vi "RDB Compose Message.vi"(8 "error in (no error)":errorcluster, 10 "RDB Reference in":T4, 11 "Settings in":T1={"UDP Receiver"=refnum, "UDP Sender"=refnum, "Valid Packet"=FALSE, "TCP"=refnum, "Network Settings"={"IP adress"="127.0.0.1", "RDB"={"Protocol"=enum."UDP", "Tx Port"=48270, "Rx Port"=10, "Buffer Size"=204800, "Timeout"=10}, "SCP"={"Protocol"=enum."TCP", "Tx Port"=48191, "Rx Port"=48191, "Buffer Size"=204800, "Timeout"=10}}, "vclient"=path "", "paeseHandle"=0, "builderHandle"=0}) -> (0 "error out":errorcluster, 2 "RDB Reference out":T4, 3 "Settings out":T1={"UDP Receiver"=refnum, "UDP Sender"=refnum, "Valid Packet"=FALSE, "TCP"=refnum, "Network Settings"={"IP adress"="127.0.0.1", "RDB"={"Protocol"=enum."UDP", "Tx Port"=48270, "Rx Port"=10, "Buffer Size"=204800, "Timeout"=10}, "SCP"={"Protocol"=enum."TCP", "Tx Port"=48191, "Rx Port"=48191, "Buffer Size"=204800, "Timeout"=10}}, "vclient"=path "", "paeseHandle"=0, "builderHandle"=0})   [LabVIEW 2023, in "RDB.lvlib"]
uses:
  RDB.lvlib
  RDB References.ctl
  DataContainer/DataContainer.lvclass
  Engine/Type/Settings.ctl
  Shared/Network Settings.ctl
  Shared/Protocol.ctl
  Shared/Vires VTD Shared.lvlib
  Engine/Vires VTD Engine.lvlib
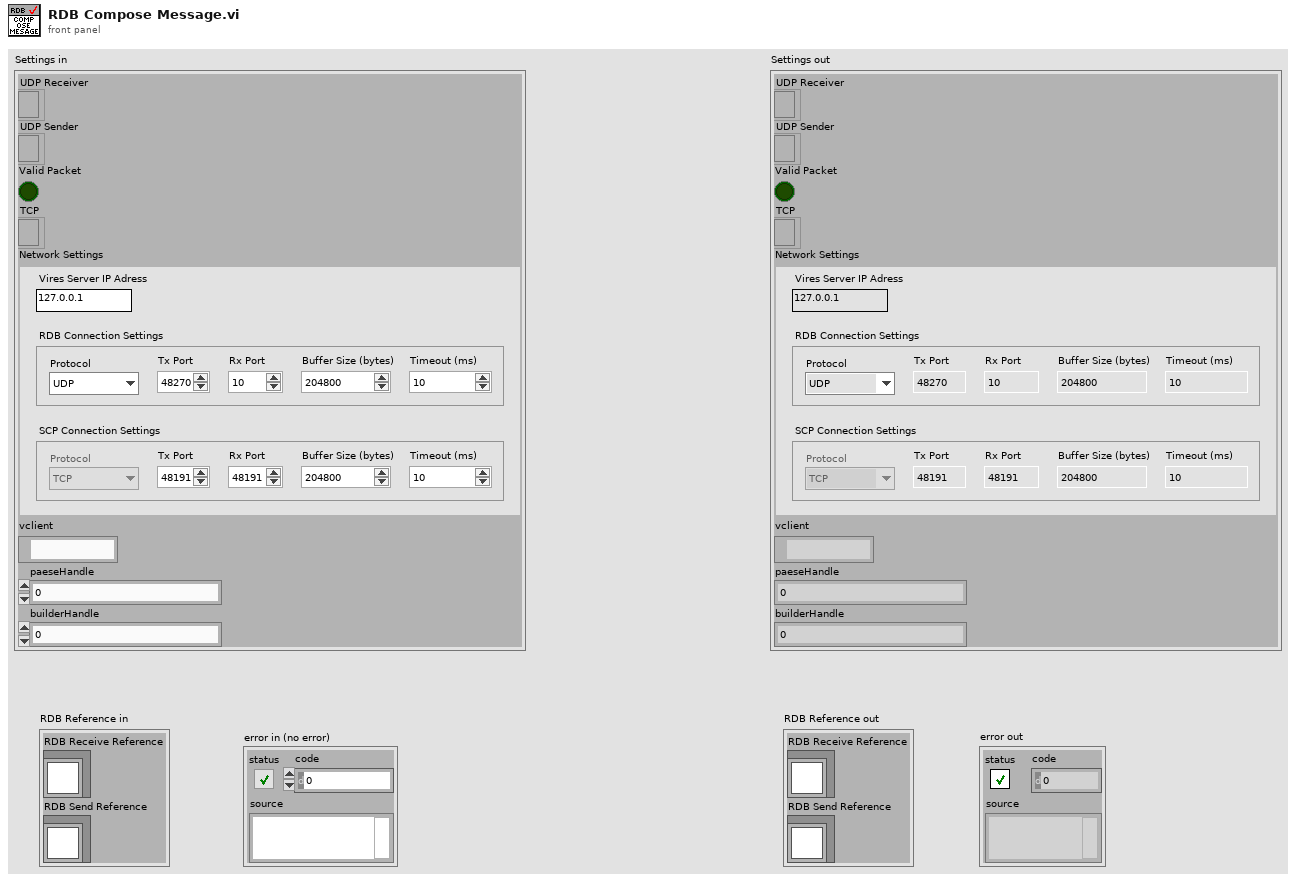
[diagram p1: front panel]
types:
  T1 = typedef "Vires VTD Engine.lvlib/Settings.ctl" = cluster{"UDP Receiver":refnum<k16>, "UDP Sender":refnum<k16>, "Valid Packet":bool, "TCP":refnum<k5>, "Network Settings":T2, "vclient":path, "paeseHandle":u64, "builderHandle":u64}
  T2 = typedef "Vires VTD Shared.lvlib/Network Settings.ctl" = cluster{"IP adress":string, "RDB":cluster{"Protocol":T3, "Tx Port":u16, "Rx Port":u16, "Buffer Size":i32, "Timeout":u16}, "SCP":cluster{"Protocol":T3, "Tx Port":u16, "Rx Port":u16, "Buffer Size":i32, "Timeout":u16}}
  T3 = typedef "Vires VTD Shared.lvlib/Protocol.ctl" = enum16{"UDP", "TCP"}
  T4 = typedef "RDB.lvlib/RDB References.ctl" = cluster{"RDB Receive Reference":refnum<class "DataContainer.lvclass">, "RDB Send Reference":refnum<class "DataContainer.lvclass">}
  T5 = typedef "XNET Frame FlexRay.ctl" = cluster{"timestamp":timestamp, "payload":u8[], "slot":u16, "type":T6, "cycle count":u8, "startup?":bool, "sync?":bool, "preamble?":bool, "ch A":bool, "ch B":bool, "echo?":bool}
  T6 = typedef "XNET Frame Type FlexRay.ctl" = u8
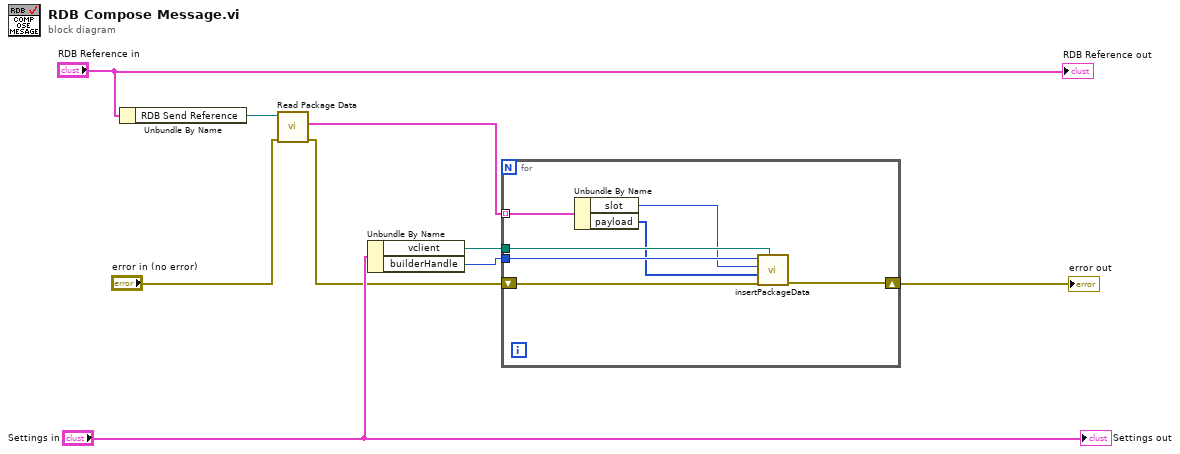
[diagram p0: block diagram]
diagram:
  n1 = Unbundle By Name("RDB Reference in") -> ("RDB Send Reference"=w4:refnum<class "DataContainer.lvclass">)
  n2 = call-dynamic "Read Package Data.vi"("error in (no error)"="error in (no error)", "DataContainer in"=w4) -> ("error out"=w1:errorcluster, "Package Data"=w3:T5[])  [unwired: 7 in, 1 out]
  n3 = Unbundle By Name("Settings in") -> ("vclient"=w6:path, "builderHandle"=w5:u64)
  n4 = for {
    shift-right: [w14] -> w9
    shift-left: w1 -> [w15]
    tunnel: w3 -> [w16] mode=indexing
    tunnel: w6 -> [w13]
    tunnel: w5 -> [w12]
    n5 = Unbundle By Name(w16) -> ("slot"=w11:u16, "payload"=w10:u8[])
    n6 = call "insertPackageData.vi"("path in"=w13, "error in (no error)"=w15, "packageData"=w10, "packageID"=w11, "builderHandle in"=w12) -> ("error out"=w14:errorcluster)  [unwired: 4 in, 2 out]
  }
  "error out" <- w9
  "RDB Reference out" <- "RDB Reference in"
  "Settings out" <- "Settings in"
